vi "Find Running Entry.vi"(8 "error in (no error)":errorcluster, 10 "Now":timestamp, 11 "Data Folder":path) -> (0 "error out":errorcluster, 2 "found?":bool, 3 "Time Entry":T1)   [LabVIEW 2024]
doc: "Looks for a running time entry - one whose End Time is 0 - in the month file of Now (UTC) and in the file of the month before. found? is FALSE when there is none; when there are several the one that started last is returned. Now is an input so the search can be tested; Time Entry Store-INI passes the current time.\n\nGenerated by: Claude"
uses:
  Rows/Time Entry.ctl
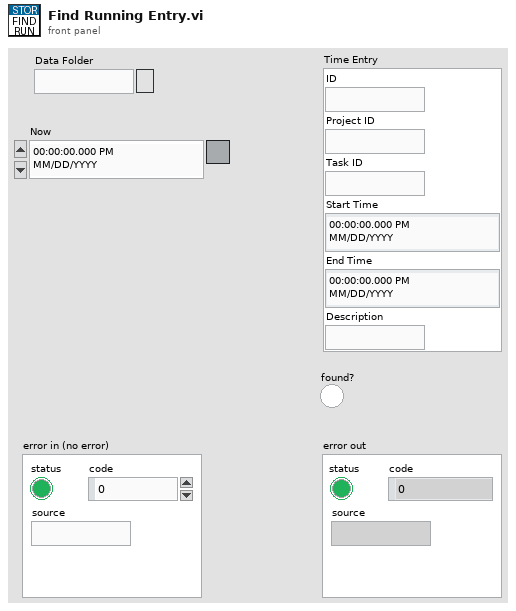
[diagram p1: front panel]
types:
  T1 = typedef "Time Entry.ctl" = cluster{"ID":string, "Project ID":string, "Task ID":string, "Start Time":timestamp, "End Time":timestamp, "Description":string}
  T2 = typedef "LVDateTimeRec.ctl" = cluster{"fractional second":dbl, "second":i32, "minute":i32, "hour":i32, "day of month":i32, "month":i32, "year":i32, "day of week":i32, "day of year":i32, "DST":i32}
  T3 = typedef "Time Entry List.ctl" = T1[]
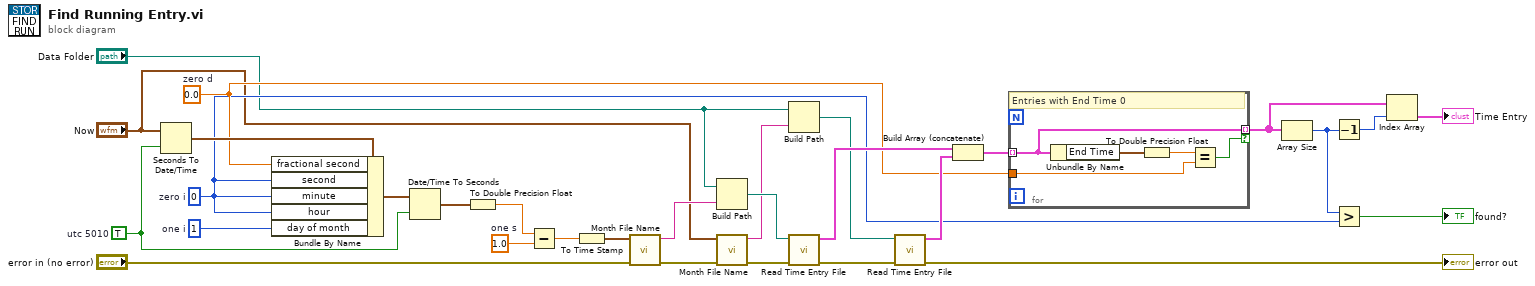
[diagram p0: block diagram]
diagram:
  w12 = 1.0  # one s
  w7 = TRUE  # utc 5010
  w6 = 0.0  # zero d
  w5 = 1  # one i
  w4 = 0  # zero i
  n1 = Seconds To Date/Time(time stamp (now)="Now", to UTC (F)=w7) -> (date time rec=w8:T2)
  n2 = Bundle By Name(cluster=w8, "fractional second"=w6, "second"=w4, "minute"=w4, "hour"=w4, "day of month"=w5) -> (w9:T2)
  n3 = Date/Time To Seconds(1:w7, 2:w9) -> (0:w10:timestamp)
  n4 = To Double Precision Float(number=w10) -> (double precision float=w11:dbl)
  n5 = Subtract(x=w11, y=w12) -> (x-y=w13:dbl)
  n6 = To Time Stamp(1:w13) -> (0:w14:timestamp)
  n7 = call "Month File Name.vi"("error in (no error)"="error in (no error)", "Start Time"=w14) -> ("error out"=w16:errorcluster, "File Name"=w15:string)  [unwired: 8 in]
  n8 = Build Path(base path="Data Folder", name or relative path=w15) -> (appended path=w19:path)
  n9 = call "Month File Name.vi"("error in (no error)"=w16, "Start Time"="Now") -> ("error out"=w18:errorcluster, "File Name"=w17:string)  [unwired: 8 in]
  n10 = Build Path(base path="Data Folder", name or relative path=w17) -> (appended path=w20:path)
  n11 = call "Read Time Entry File.vi"("error in (no error)"=w18, "File Path"=w19) -> ("error out"=w22:errorcluster, "Time Entries"=w21:T3)  [unwired: 6 in, 2 out]
  n12 = call "Read Time Entry File.vi"("error in (no error)"=w22, "File Path"=w20) -> ("error out"=→"error out":errorcluster, "Time Entries"=w23:T3)  [unwired: 6 in, 2 out]
  n13 = Build Array (concatenate)(w21, w23) -> (w25:T3)
  n14 = for {
    tunnel: w6 -> [w32]
    tunnel: w25 -> [w31] mode=indexing
    tunnel: [w31] -> w26 mode=indexing if=w35
    # "Entries with End Time 0"
    n15 = Unbundle By Name(w31) -> ("End Time"=w33:timestamp)
    n16 = To Double Precision Float(number=w33) -> (double precision float=w34:dbl)
    n17 = Equal?(x=w34, y=w32) -> (x = y?=w35:bool)
  }
  n18 = Array Size(array=w26) -> (size(s)=w27:i32)
  n19 = Decrement(x=w27) -> (x-1=w29:i32)
  n20 = Greater?(x=w27, y=w4) -> (0:→"found?":bool)
  n21 = Index Array(array=w26, index=w29) -> (element=→"Time Entry":T1)
